vi "Configuration Parse.vi"(8 "error in":errorcluster, 11 "Measurement Configuration":T3={"Automation Test"=FALSE, "Power sequencing file path"="", "SMU name"="", "SMU channel"="0", "RFSG name"="5842", "RFSG port"="port1", "RFSG attenuation mode"=enum."<None>", "RFSG external attenuation (dB)"=0.0, "RFSG s-parameters orientation"=enum."Port1 Towards DUT", "RFSG s2p file path"="", "RFmx name"="5842", "RFmx port"="port2", "RFmx attenuation mode"=enum."<None>", "RFmx external attenuation (dB)"=0.0, "RFmx attenuation path name"="", "RFmx s-parameters orientation"=enum."Port1 Towards DUT", "RFmx attenuation s2p path name"="", "RFmx s2p file path"="", "Compression_Expected DUT Gain (dB)"=17.5, "Compression_Max Linear Range (dBm)"=-10.0, "Compression_Compression Point (dB)"=1.0, "Compression_Target Pin (dBm)"=1.0, "Compression_RFSG Frequency Start (Hz)"=6000000000.0, "Compression_RFSG Frequency Stop (Hz)"=18000000000.0, "Compression_RFSG Number of Frequency Step"=11, "Compression_RFSG Power Start (dBm)"=-20.0, "Compression_RFSG Power Stop(dBm)"=4.0, "Compression_RFSG Power Step Size (dB)"=1.0, "Compression_RBW (Hz)"=5000000.0, "Compression_RF Measurement Interval (s)"=5e-05, "Compression_DC Measurement Interval (s)"=5e-05, "Compression_Stimulus Mode"=enum."Constant Power and RF", "CP_CW_DC Source Delay (s)"=0.0, "CP_PRF_DC Source Delay (s)"=0.0, "CP_PRF_RFmx Trigger Delay (s)"=0.0, "CP_PRF_RF Pulse Width (s)"=0.0001, "CP_PRF_PRI (s)"=0.001, "PP_PRF_DC Source Delay (s)"=0.0, "PP_PRF_RFmx Trigger Delay (s)"=0.0, "PP_PRF_RF Pulse Width (s)"=0.0001, "PP_PRF_PRI (s)"=0.001, "PP_PRF_DC Pulse Width (s)"=0.0008, "PP_PRF_ON Current Limit (A)"=2.0, "PP_PRF_Bias Voltage Level (V)"=0.0, "PP_PRF_Bias Current Limit (A)"=0.2, "Power sequecing file validity check"=FALSE} {"Compression_Target Pin (dBm)" format="%#pdBm"; "PP_PRF_Bias Current Limit (A)" format="%#pA"; "PP_PRF_Bias Voltage Level (V)" format="%#pV"; "PP_PRF_ON Current Limit (A)" format="%#pA"; "PP_PRF_DC Pulse Width (s)" format="%#ps"; "PP_PRF_PRI (s)" format="%#ps"; "PP_PRF_RF Pulse Width (s)" format="%#ps"; "PP_PRF_RFmx Trigger Delay (s)" format="%#ps"; "PP_PRF_DC Source Delay (s)" format="%#ps"; "CP_PRF_PRI (s)" format="%#ps"; "CP_PRF_RF Pulse Width (s)" format="%#ps"; "CP_PRF_RFmx Trigger Delay (s)" format="%#ps"; "CP_PRF_DC Source Delay (s)" format="%#ps"; "CP_CW_DC Source Delay (s)" format="%#ps"; "Compression_DC Measurement Interval (s)" format="%#ps"; "Compression_RF Measurement Interval (s)" format="%#ps"; "RFmx external attenuation (dB)" format="%.2f"; "RFSG external attenuation (dB)" format="%.2f"}) -> (0 "error out":errorcluster, 1 "RFmx Settings":T5 {"Attenuation"."s2p File"."RFmx S-Parameters Orientation" items=["Port1 Towards DUT"=24000, "Port2 Towards DUT"=24001]; "Attenuation"."Constant Attenuation"."RFmx External Attenuation (dB)" format="%.2f"}, 2 "RFSG Settings":T4 {"Attenuation"."s2p File"."RFSG S-parameters Orientation" items=["Port1 Towards DUT"=24000, "Port2 Towards DUT"=24001]; "Attenuation"."Contant Attenuation"."RFSG External Attenuation (dB)" format="%.2f"}, 3 "Test Configuration":T2={"Expected DUT Gain (dB)"=0.0, "Max Linear Range (dBm)"=0.0, "Compression Point (dB)"=0.0, "Pout at Pin (dBm)"=1.0, "RFSG Frequency Start (Hz)"=0.0, "RFSG Frequency Stop (Hz)"=0.0, "RFSG Number of Frequency Step"=0, "Power Start (dBm)"=0.0, "Power Stop(dBm)"=0.0, "Power Step Size (dB)"=0.0, "RBW (Hz)"=0.0, "Modes"={"RF Measurement Interval (s)"=0.001, "DC Measurement Interval (s)"=0.0, "Power Stimulus Mode"=enum."Constant Power and RF", "CP_CW_DC Source Delay (s)"=0.0002, "CP_PRF_DC Source Delay (s)"=0.0, "CP_PRF_RFmx Trigger Delay (s)"=0.2, "CP_PRF_RF Pulse Width (s)"=0.0009, "CP_PRF_PRI (s)"=0.015, "PP_PRF_DC Source Delay (s)"=0.0, "PP_PRF_RFmx Trigger Delay (s)"=0.0, "PP_PRF_RF Pulse Width (s)"=0.0, "PP_PRF_PRI (s)"=0.0, "PP_PRF_DC Pulse Width (s)"=0.0008, "PP_PRF_Bias Voltage Level (V)"=0.0, "PP_PRF_Bias Current Limit (A)"=0.2}} {"Pout at Pin (dBm)" format="%#pdBm"; "Modes"."PP_PRF_Bias Current Limit (A)" format="%#pA"; "Modes"."PP_PRF_Bias Voltage Level (V)" format="%#pV"; "Modes"."PP_PRF_DC Pulse Width (s)" format="%#ps"; "Modes"."PP_PRF_PRI (s)" format="%#ps"; "Modes"."PP_PRF_RF Pulse Width (s)" format="%#ps"; "Modes"."PP_PRF_RFmx Trigger Delay (s)" format="%#ps"; "Modes"."PP_PRF_DC Source Delay (s)" format="%#ps"; "Modes"."CP_PRF_PRI (s)" format="%#ps"; "Modes"."CP_PRF_RF Pulse Width (s)" format="%#ps"; "Modes"."CP_PRF_RFmx Trigger Delay (s)" format="%#ps"; "Modes"."CP_PRF_DC Source Delay (s)" format="%#ps"; "Modes"."CP_CW_DC Source Delay (s)" format="%#ps"; "Modes"."DC Measurement Interval (s)" format="%#_6p"; "RFSG Frequency Stop (Hz)" format="%#_6p"; "Power Start (dBm)" format="%#_6p"; "Power Stop(dBm)" format="%#_6p"; "RFSG Frequency Start (Hz)" format="%#_6p"; "Expected DUT Gain (dB)" step=1.0 format="%#_6p"}, 5 "SMU Settings":T1={"SMU Name"="PXI1Slot15", "SMU Channel"="2", "IDD Current Limit (A)"=0.0})   [LabVIEW 2023, in "FPT_Compression.lvclass"]
uses:
  FPT_Compression.lvclass
  Measurement/Controls/RFmx Config - Compression.ctl
  Measurement/Controls/RFSG Config - Compression.ctl
  Measurement Configuration.ctl
  Measurement/Controls/Test Config - Compression.ctl
  Measurement/Controls/SMU Config - Compression.ctl
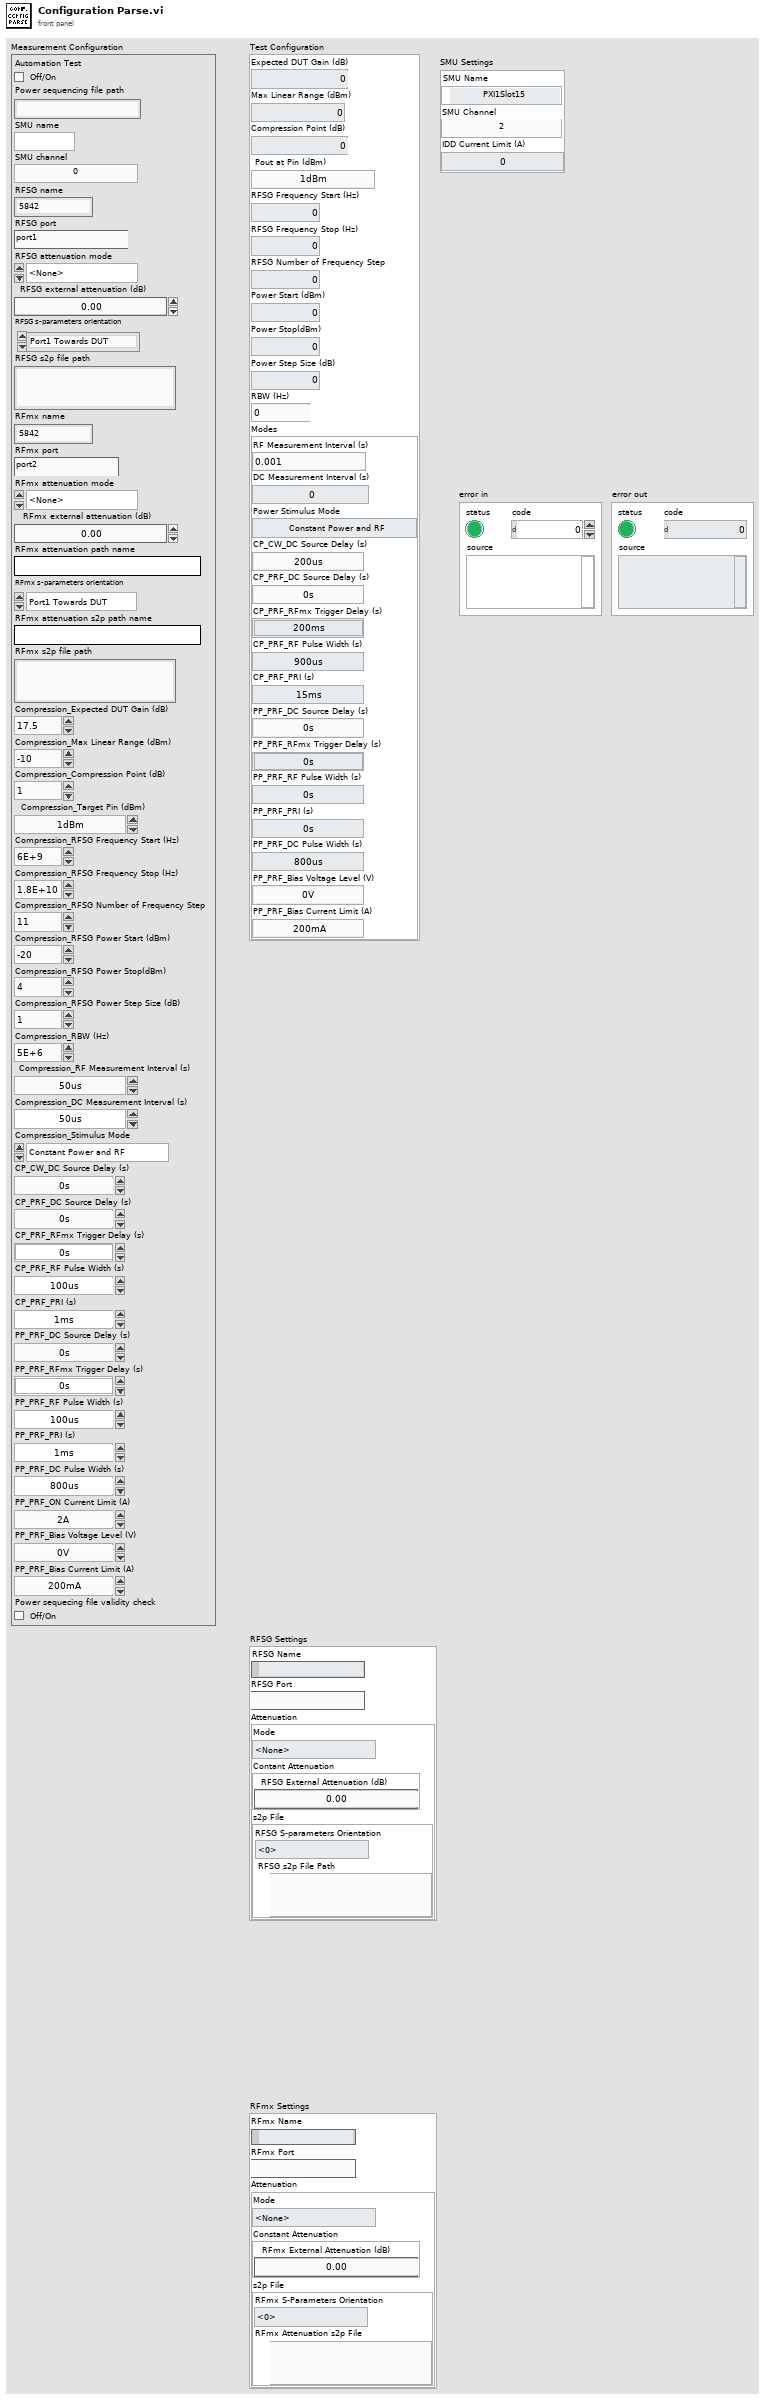
[diagram p1: front panel]
types:
  T1 = typedef "SMU Config - Compression.ctl" = cluster{"SMU Name":refnum<k15>, "SMU Channel":string, "IDD Current Limit (A)":dbl}
  T2 = typedef "Test Config - Compression.ctl" = cluster{"Expected DUT Gain (dB)":dbl, "Max Linear Range (dBm)":dbl, "Compression Point (dB)":dbl, "Pout at Pin (dBm)":dbl, "RFSG Frequency Start (Hz)":dbl, "RFSG Frequency Stop (Hz)":dbl, "RFSG Number of Frequency Step":i32, "Power Start (dBm)":dbl, "Power Stop(dBm)":dbl, "Power Step Size (dB)":dbl, "RBW (Hz)":dbl, "Modes":cluster{"RF Measurement Interval (s)":dbl, "DC Measurement Interval (s)":dbl, "Power Stimulus Mode":enum16{"Constant Power and RF", "Constant Power and Pulsed RF", "Pulsed Power and RF"}, "CP_CW_DC Source Delay (s)":dbl, "CP_PRF_DC Source Delay (s)":dbl, "CP_PRF_RFmx Trigger Delay (s)":dbl, "CP_PRF_RF Pulse Width (s)":dbl, "CP_PRF_PRI (s)":dbl, "PP_PRF_DC Source Delay (s)":dbl, "PP_PRF_RFmx Trigger Delay (s)":dbl, "PP_PRF_RF Pulse Width (s)":dbl, "PP_PRF_PRI (s)":dbl, "PP_PRF_DC Pulse Width (s)":dbl, "PP_PRF_Bias Voltage Level (V)":dbl, "PP_PRF_Bias Current Limit (A)":dbl}}
  T3 = typedef "FPT_Compression.lvclass/Measurement Configuration.ctl" = cluster{"Automation Test":bool, "Power sequencing file path":string, "SMU name":string, "SMU channel":string, "RFSG name":string, "RFSG port":string, "RFSG attenuation mode":enum32{"<None>", "Constant Attenuation", "s2p File"}, "RFSG external attenuation (dB)":dbl, "RFSG s-parameters orientation":enum32{"Port1 Towards DUT", "Port2 Towards DUT"}, "RFSG s2p file path":string, "RFmx name":string, "RFmx port":string, "RFmx attenuation mode":enum32{"<None>", "Constant Attenuation", "s2p File"}, "RFmx external attenuation (dB)":dbl, "RFmx attenuation path name":string, "RFmx s-parameters orientation":enum32{"Port1 Towards DUT", "Port2 Towards DUT"}, "RFmx attenuation s2p path name":string, "RFmx s2p file path":string, "Compression_Expected DUT Gain (dB)":dbl, "Compression_Max Linear Range (dBm)":dbl, "Compression_Compression Point (dB)":dbl, "Compression_Target Pin (dBm)":dbl, "Compression_RFSG Frequency Start (Hz)":dbl, "Compression_RFSG Frequency Stop (Hz)":dbl, "Compression_RFSG Number of Frequency Step":i32, "Compression_RFSG Power Start (dBm)":dbl, "Compression_RFSG Power Stop(dBm)":dbl, "Compression_RFSG Power Step Size (dB)":dbl, "Compression_RBW (Hz)":dbl, "Compression_RF Measurement Interval (s)":dbl, "Compression_DC Measurement Interval (s)":dbl, "Compression_Stimulus Mode":enum32{"Constant Power and RF", "Constant Power and Pulsed RF", "Pulsed Power and RF"}, "CP_CW_DC Source Delay (s)":dbl, "CP_PRF_DC Source Delay (s)":dbl, "CP_PRF_RFmx Trigger Delay (s)":dbl, "CP_PRF_RF Pulse Width (s)":dbl, "CP_PRF_PRI (s)":dbl, "PP_PRF_DC Source Delay (s)":dbl, "PP_PRF_RFmx Trigger Delay (s)":dbl, "PP_PRF_RF Pulse Width (s)":dbl, "PP_PRF_PRI (s)":dbl, "PP_PRF_DC Pulse Width (s)":dbl, "PP_PRF_ON Current Limit (A)":dbl, "PP_PRF_Bias Voltage Level (V)":dbl, "PP_PRF_Bias Current Limit (A)":dbl, "Power sequecing file validity check":bool}
  T4 = typedef "RFSG Config - Compression.ctl" = cluster{"RFSG Name":refnum<k15>, "RFSG Port":string, "Attenuation":cluster{"Mode":enum32{"<None>", "Constant Attenuation", "s2p File"}, "Contant Attenuation":cluster{"RFSG External Attenuation (dB)":dbl}, "s2p File":cluster{"RFSG S-parameters Orientation":i32, "RFSG s2p File Path":path}}}
  T5 = typedef "RFmx Config - Compression.ctl" = cluster{"RFmx Name":refnum<k15>, "RFmx Port":string, "Attenuation":cluster{"Mode":enum32{"<None>", "Constant Attenuation", "s2p File"}, "Constant Attenuation":cluster{"RFmx External Attenuation (dB)":dbl}, "s2p File":cluster{"RFmx S-Parameters Orientation":i32, "RFmx Attenuation s2p File":path}}}
  T6 = enum32{"<None>", "Constant Attenuation", "s2p File"}
  T7 = enum32{"Constant Power and RF", "Constant Power and Pulsed RF", "Pulsed Power and RF"}
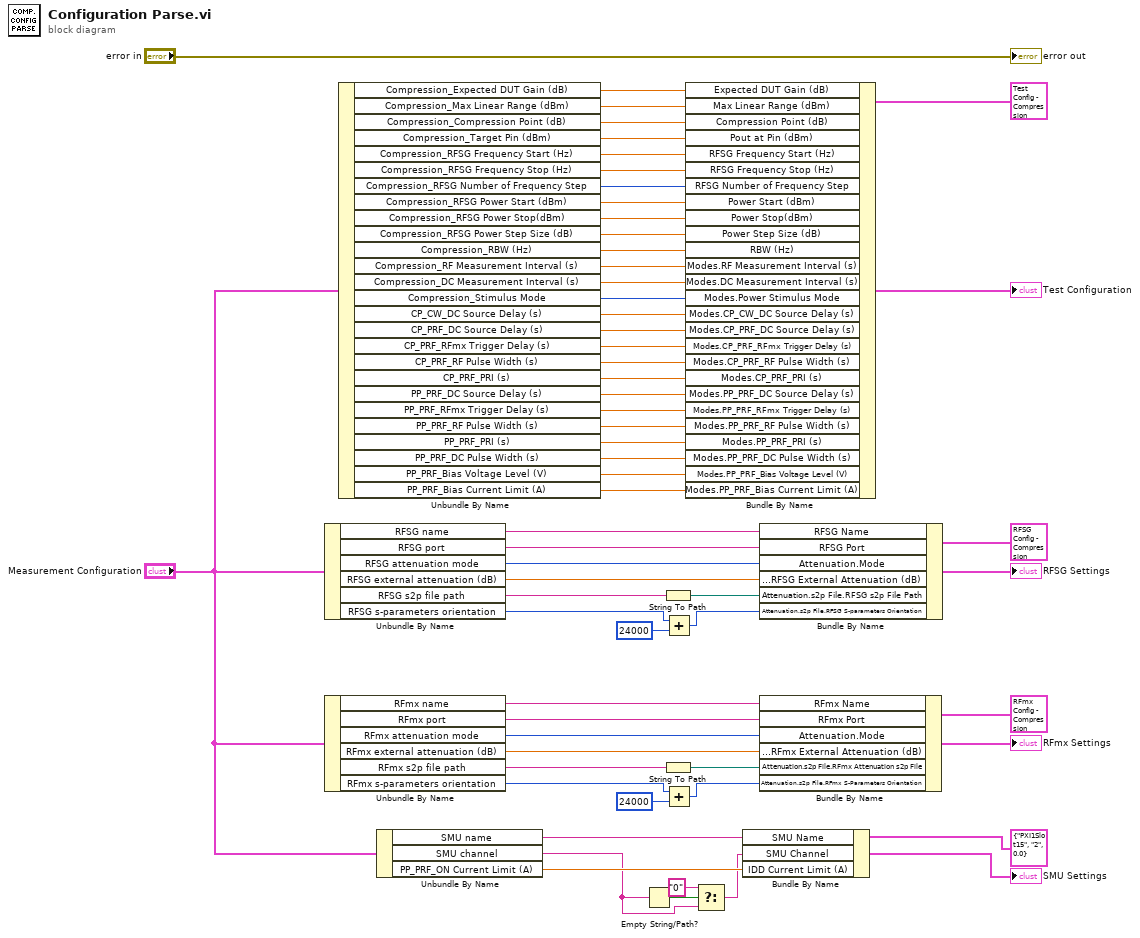
[diagram p0: block diagram]
diagram:
  n1 = Unbundle By Name("Measurement Configuration") -> ("RFSG name"=w48:string, "RFSG port"=w57:string, "RFSG attenuation mode"=w42:T6, "RFSG external attenuation (dB)"=w49:dbl, "RFSG s2p file path"=w53:string, "RFSG s-parameters orientation"=w41:enum32{"Port1 Towards DUT", "Port2 Towards DUT"})
  n2 = Unbundle By Name("Measurement Configuration") -> ("RFmx name"=w51:string, "RFmx port"=w58:string, "RFmx attenuation mode"=w43:T6, "RFmx external attenuation (dB)"=w52:dbl, "RFmx s2p file path"=w56:string, "RFmx s-parameters orientation"=w37:enum32{"Port1 Towards DUT", "Port2 Towards DUT"})
  n3 = Unbundle By Name("Measurement Configuration") -> ("Compression_Expected DUT Gain (dB)"=w20:dbl, "Compression_Max Linear Range (dBm)"=w19:dbl, "Compression_Compression Point (dB)"=w18:dbl, "Compression_Target Pin (dBm)"=w17:dbl, "Compression_RFSG Frequency Start (Hz)"=w16:dbl, "Compression_RFSG Frequency Stop (Hz)"=w15:dbl, "Compression_RFSG Number of Frequency Step"=w14:i32, "Compression_RFSG Power Start (dBm)"=w13:dbl, "Compression_RFSG Power Stop(dBm)"=w12:dbl, "Compression_RFSG Power Step Size (dB)"=w11:dbl, "Compression_RBW (Hz)"=w10:dbl, "Compression_RF Measurement Interval (s)"=w9:dbl, "Compression_DC Measurement Interval (s)"=w8:dbl, "Compression_Stimulus Mode"=w1:T7, "CP_CW_DC Source Delay (s)"=w26:dbl, "CP_PRF_DC Source Delay (s)"=w25:dbl, "CP_PRF_RFmx Trigger Delay (s)"=w24:dbl, "CP_PRF_RF Pulse Width (s)"=w23:dbl, "CP_PRF_PRI (s)"=w22:dbl, "PP_PRF_DC Source Delay (s)"=w21:dbl, "PP_PRF_RFmx Trigger Delay (s)"=w7:dbl, "PP_PRF_RF Pulse Width (s)"=w6:dbl, "PP_PRF_PRI (s)"=w5:dbl, "PP_PRF_DC Pulse Width (s)"=w4:dbl, "PP_PRF_Bias Voltage Level (V)"=w3:dbl, "PP_PRF_Bias Current Limit (A)"=w2:dbl)
  n4 = Unbundle By Name("Measurement Configuration") -> ("SMU name"=w32:string, "SMU channel"=w28:string, "PP_PRF_ON Current Limit (A)"=w31:dbl)
  n5 = Empty String/Path?(string/path=w28) -> (empty?=w30:bool)
  n6 = String To Path(string=w53) -> (path=w54:path)
  n7 = String To Path(string=w56) -> (path=w55:path)
  n8 = Add(x=w41, y=u32 24000) -> (x+y=w39:u32)
  n9 = Add(x=w37, y=u32 24000) -> (x+y=w36:u32)
  n10 = Bundle By Name(cluster=T2 {"Expected DUT Gain (dB)"=0.0, "Max Linear Range (dBm)"=0.0, "Compression Point (dB)"=0.0, "Pout at Pin (dBm)"=1.0, "RFSG Frequency Start (Hz)"=0.0, "RFSG Frequency Stop (Hz)"=0.0, "RFSG Number of Frequency Step"=0, "Power Start (dBm)"=0.0, "Power Stop(dBm)"=0.0, "Power Step Size (dB)"=0.0, "RBW (Hz)"=0.0, "Modes"={"RF Measurement Interval (s)"=0.001, "DC Measurement Interval (s)"=0.0, "Power Stimulus Mode"=enum."Constant Power and RF", "CP_CW_DC Source Delay (s)"=0.0002, "CP_PRF_DC Source Delay (s)"=0.0, "CP_PRF_RFmx Trigger Delay (s)"=0.2, "CP_PRF_RF Pulse Width (s)"=0.0009, "CP_PRF_PRI (s)"=0.015, "PP_PRF_DC Source Delay (s)"=0.0, "PP_PRF_RFmx Trigger Delay (s)"=0.0, "PP_PRF_RF Pulse Width (s)"=0.0, "PP_PRF_PRI (s)"=0.0, "PP_PRF_DC Pulse Width (s)"=0.0008, "PP_PRF_Bias Voltage Level (V)"=0.0, "PP_PRF_Bias Current Limit (A)"=0.2}} ("Test Configuration"), "Expected DUT Gain (dB)"=w20, "Max Linear Range (dBm)"=w19, "Compression Point (dB)"=w18, "Pout at Pin (dBm)"=w17, "RFSG Frequency Start (Hz)"=w16, "RFSG Frequency Stop (Hz)"=w15, "RFSG Number of Frequency Step"=w14, "Power Start (dBm)"=w13, "Power Stop(dBm)"=w12, "Power Step Size (dB)"=w11, "RBW (Hz)"=w10, "Modes.RF Measurement Interval (s)"=w9, "Modes.DC Measurement Interval (s)"=w8, "Modes.Power Stimulus Mode"=w1, "Modes.CP_CW_DC Source Delay (s)"=w26, "Modes.CP_PRF_DC Source Delay (s)"=w25, "Modes.CP_PRF_RFmx Trigger Delay (s)"=w24, "Modes.CP_PRF_RF Pulse Width (s)"=w23, "Modes.CP_PRF_PRI (s)"=w22, "Modes.PP_PRF_DC Source Delay (s)"=w21, "Modes.PP_PRF_RFmx Trigger Delay (s)"=w7, "Modes.PP_PRF_RF Pulse Width (s)"=w6, "Modes.PP_PRF_PRI (s)"=w5, "Modes.PP_PRF_DC Pulse Width (s)"=w4, "Modes.PP_PRF_Bias Voltage Level (V)"=w3, "Modes.PP_PRF_Bias Current Limit (A)"=w2) -> (→"Test Configuration":T2)
  n11 = Select(t="0", s=w30, f=w28) -> (s? t:f=w29:string)
  n12 = Bundle By Name(cluster=T1 {"SMU Name"="PXI1Slot15", "SMU Channel"="2", "IDD Current Limit (A)"=0.0} ("SMU Settings"), "SMU Name"=w32, "SMU Channel"=w29, "IDD Current Limit (A)"=w31) -> (→"SMU Settings":T1)
  n13 = Bundle By Name(cluster=T4 {"RFSG Name"="5842_0", "RFSG Port"="", "Attenuation"={"Mode"=enum."Constant Attenuation", "Contant Attenuation"={"RFSG External Attenuation (dB)"=2.0}, "s2p File"={"RFSG S-parameters Orientation"=24000, "RFSG s2p File Path"=path ""}}} ("RFSG Settings"), "RFSG Name"=w48, "RFSG Port"=w57, "Attenuation.Mode"=w42, "Attenuation.Contant Attenuation.RFSG External Attenuation (dB)"=w49, "Attenuation.s2p File.RFSG s2p File Path"=w54, "Attenuation.s2p File.RFSG S-parameters Orientation"=w39) -> (→"RFSG Settings":T4)
  n14 = Bundle By Name(cluster=T5 {"RFmx Name"="5842_0", "RFmx Port"="", "Attenuation"={"Mode"=enum."Constant Attenuation", "Constant Attenuation"={"RFmx External Attenuation (dB)"=1.2}, "s2p File"={"RFmx S-Parameters Orientation"=24000, "RFmx Attenuation s2p File"=path ""}}} ("RFmx Settings"), "RFmx Name"=w51, "RFmx Port"=w58, "Attenuation.Mode"=w43, "Attenuation.Constant Attenuation.RFmx External Attenuation (dB)"=w52, "Attenuation.s2p File.RFmx Attenuation s2p File"=w55, "Attenuation.s2p File.RFmx S-Parameters Orientation"=w36) -> (→"RFmx Settings":T5)
  "error out" <- "error in"
